vi "Startup.vi"(6 "LabVIEW Web Service":refnum<class "Web Service.lvclass"> caption="LabVIEW Web Serivce") -> ()   [LabVIEW 2017]
uses:
  <vilib>/wsapi/Web Service.lvclass
  Example/MockTool.lvclass
  C:/Users/Jan/Projects/opentool-labview/Server/ITool/ITool.lvclass
  ITool/ITool.lvclass
panel:
  out "daemon error":string
  out "id":string
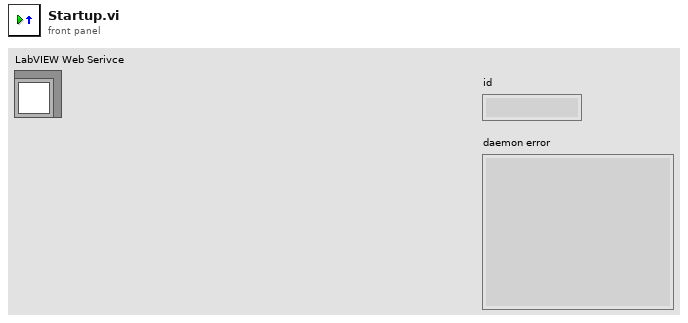
[diagram p1: front panel]
types:
  T1 = cluster{"DaemonUrl":string, "Host":string, "Port":i32, "Prefix":string}
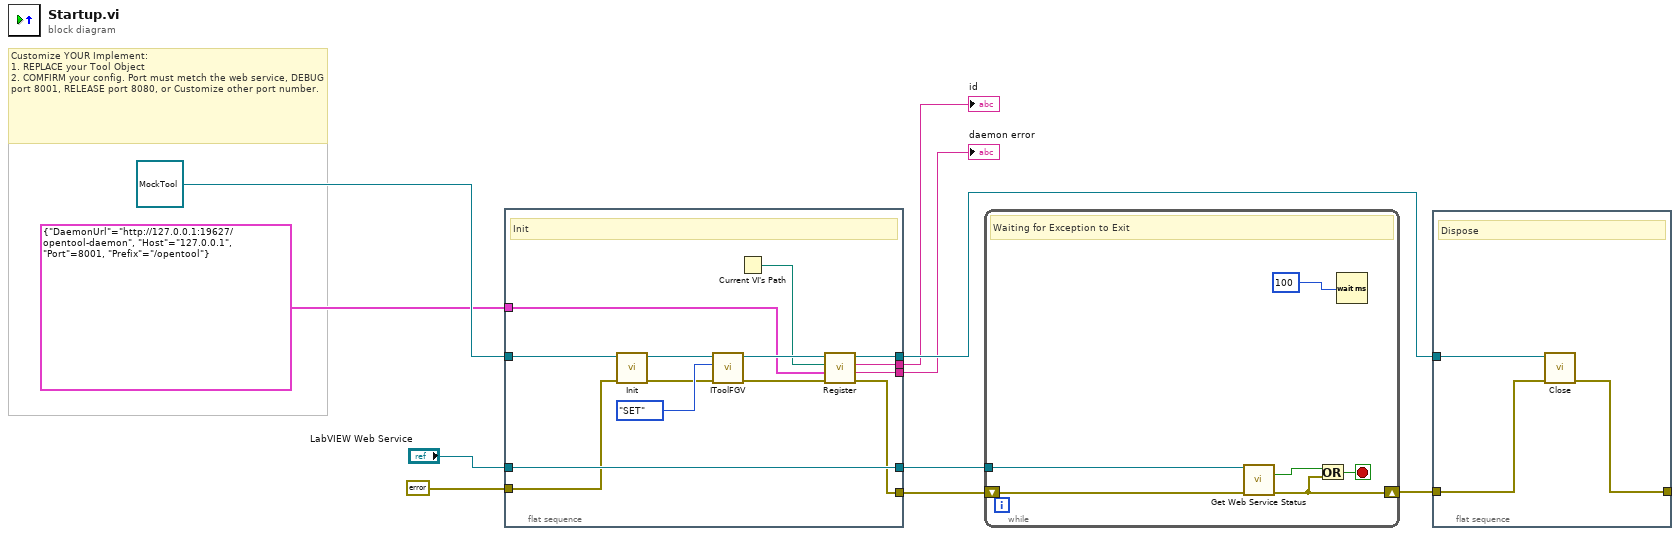
[diagram p0: block diagram]
diagram:
  # "Customize YOUR Implement:\n1. REPLACE your Tool Object\n2. COMFIRM your config. Port must metch the web service, DEBUG port 8001, RELEASE port 8080, or Customize other port number."
  n1 = flat-sequence {
    tunnel: "LabVIEW Web Service" -> [w23]
    tunnel: [w23] -> w10
    tunnel: [w16] -> w9
    tunnel: errorcluster {"status"=FALSE, "code"=0, "source"=""} ("error constant") -> [w22]
    tunnel: refnum<class "MockTool.lvclass"> refnum ("MockTool.lvclass") -> [w19]
    tunnel: [w15] -> w4
    tunnel: T1 {"DaemonUrl"="http://127.0.0.1:19627/opentool-daemon", "Host"="127.0.0.1", "Port"=8001, "Prefix"="/opentool"} -> [w14]
    tunnel: [w12] -> w2
    tunnel: [w11] -> w1
    frame #0 {
      # "Init"
      n2 = call-dynamic "Init.vi"("error in (no error)"=w22, "Tool in"=w19) -> ("error out"=w17:errorcluster, "Tool out"=w21:refnum<class "MockTool.lvclass">)  [unwired: 8 in]
      n3 = call "IToolFGV.vi"("Action"=enum16{"GET", "SET"}."SET", "ITool.lvclass in"=w21) -> ("ITool.lvclass out"=w18:refnum<class "ITool.lvclass">)  [unwired: 9 in]
      n4 = Current VI's Path() -> (path=w13:path)
      n5 = call "Register.vi"("error in (no error)"=w17, "ServerInfo"=w14, "StartupFile"=w13, "ITool.lvclass in"=w18) -> ("error out"=w16:errorcluster, "DaemonError"=w11:string, "Id"=w12:string, "ITool.lvclass out"=w15:refnum<class "ITool.lvclass">)  [unwired: 4 in]
    }
  }
  n6 = while {
    tunnel: w10 -> [w28]
    shift-right: [w25] -> w7
    shift-left: w9 -> [w26]
    stop <- w27 stop-if-true
    # "Waiting for Exception to Exit"
    n7 = call <vilib>:"Get Web Service Status.vi"("LabVIEW Web Service"=w28, "error in (no error)"=w26) -> ("service stopping?"=w29:bool, "error out"=w25:errorcluster)  [unwired: 11 in, 1 out]
    n8 = Or(x=w29, y=w25) -> (x .or. y?=w27:bool)
    n9 = Wait (ms)(milliseconds to wait=u32 100) -> ()  [unwired: 1 out]
  }
  n10 = flat-sequence {
    tunnel: [w31] -> _
    tunnel: w7 -> [w32]
    tunnel: w4 -> [w30]
    frame #0 {
      # "Dispose"
      n11 = call-dynamic "Close.vi"("error in (no error)"=w32, "Tool in"=w30) -> ("error out"=w31:errorcluster)  [unwired: 8 in, 1 out]
    }
  }
  "id" <- w2
  "daemon error" <- w1
